vi "GenerateArmMotionProfilePoints.vi"(3 "MotionProfileGeneratorParameters":T4={"Trajectory Point Interval (ms)"=10, "Maximum Travel Speed (units/s)"=0.0, "Velocity Ramp Time (ms)"=0.0, "Acceleration Ramp Time (ms)"=1.0} {"Acceleration Ramp Time (ms)" min=1.0; "Velocity Ramp Time (ms)" min=1.0; "Maximum Travel Speed (units/s)" min=0.0; "Trajectory Point Interval (ms)" items=["TrajectoryDuration_0ms"=0, "TrajectoryDuration_5ms"=5, "TrajectoryDuration_10ms"=10, "TrajectoryDuration_20ms"=20, "TrajectoryDuration_30ms"=30, "TrajectoryDuration_40ms"=40, "TrajectoryDuration_50ms"=50, "TrajectoryDuration_100ms"=100]}, 4 "PathDistance":dbl, 5 "ArmPathIn":T1[](array[typedef]), 6 "IndexedPathLength":dbl[](array[numeric])) -> (0 "ArmPathOut":T1[](array[typedef]), 1 "ExtendPath":T2[](array[typedef]) {"Time (ms)" items=["TrajectoryDuration_0ms"=0, "TrajectoryDuration_5ms"=5, "TrajectoryDuration_10ms"=10, "TrajectoryDuration_20ms"=20, "TrajectoryDuration_30ms"=30, "TrajectoryDuration_40ms"=40, "TrajectoryDuration_50ms"=50, "TrajectoryDuration_100ms"=100]}, 2 "RotatePath":T2[](array[typedef]) {"Time (ms)" items=["TrajectoryDuration_0ms"=0, "TrajectoryDuration_5ms"=5, "TrajectoryDuration_10ms"=10, "TrajectoryDuration_20ms"=20, "TrajectoryDuration_30ms"=30, "TrajectoryDuration_40ms"=40, "TrajectoryDuration_50ms"=50, "TrajectoryDuration_100ms"=100]})   [LabVIEW 2017]
uses:
  TypeDefs/ArmCoordinate.ctl
  General/MotionProfiling/TypeDefs/MotionProfileGeneratorParams.ctl
  <vilib>/Rock Robotics/WPI/ThirdParty/Phoenix-LabVIEW/Motor Controller/Controls/CTRE_Phoenix_MotorControl_TrajectoryPointTimeDur.ctl
  General/MotionProfiling/TypeDefs/TrajectoryPoint.ctl
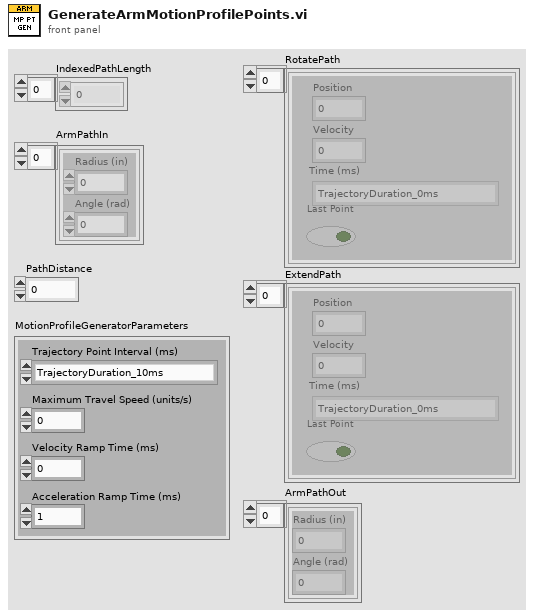
[diagram p1: front panel]
types:
  T1 = typedef "ArmCoordinate.ctl" = cluster{"Radius (in)":dbl, "Angle (rad)":dbl}
  T2 = typedef "TrajectoryPoint.ctl" = cluster{"Position ":dbl, "Velocity ":dbl, "Time (ms)":T3, "Last Point":bool}
  T3 = typedef "CTRE_Phoenix_MotorControl_TrajectoryPointTimeDur.ctl" = i32
  T4 = typedef "MotionProfileGeneratorParams.ctl" = cluster{"Trajectory Point Interval (ms)":T3, "Maximum Travel Speed (units/s)":dbl, "Velocity Ramp Time (ms)":dbl, "Acceleration Ramp Time (ms)":dbl}
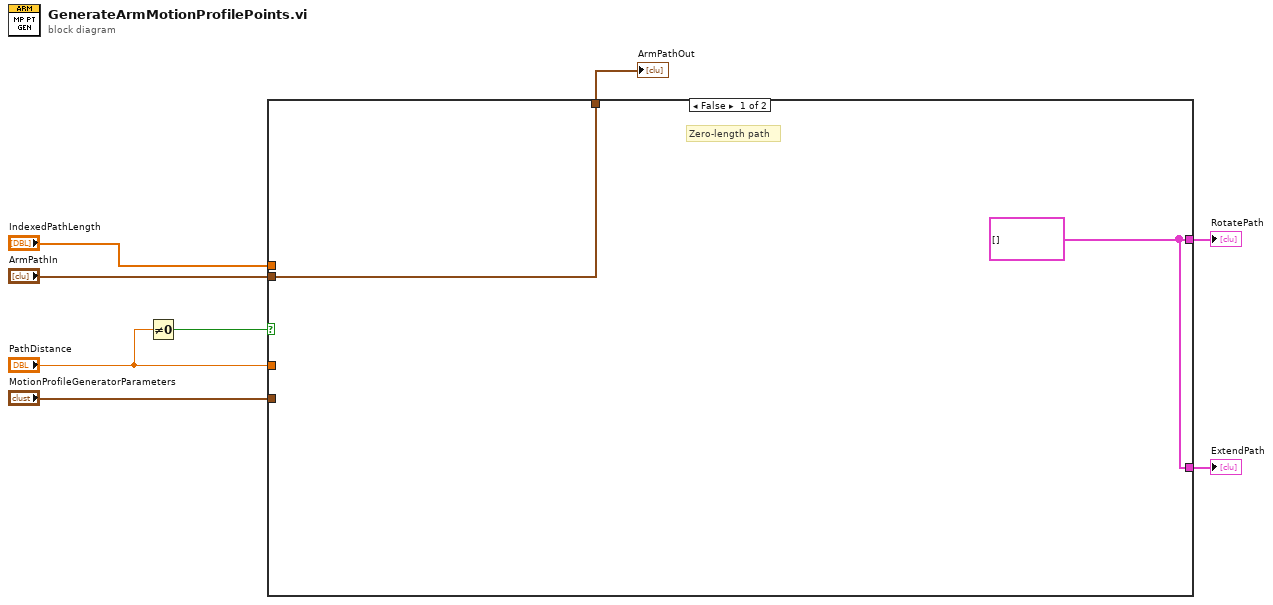
[diagram p0: block diagram]
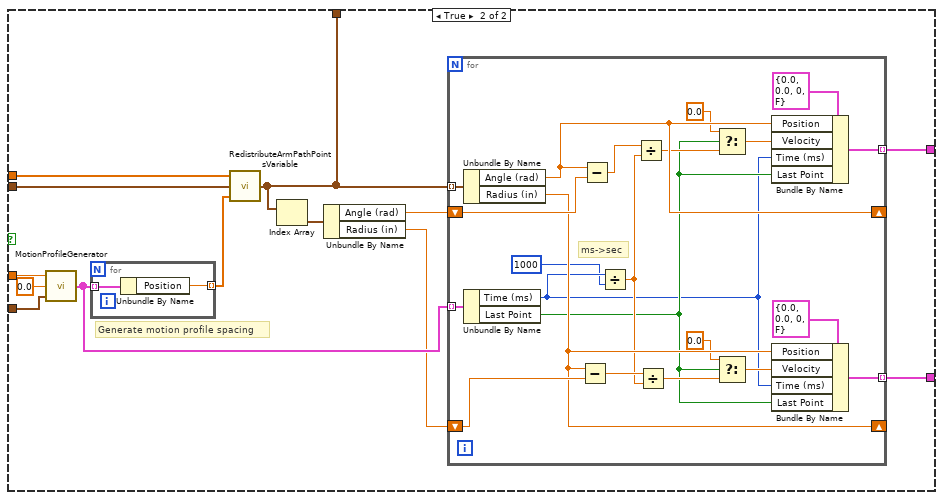
[diagram p2: hidden frame]
diagram:
  n1 = Not Equal To 0?(x="PathDistance") -> (x != 0?=w1:bool)
  n2 = case shown="False" w1 {
    tunnel: "ArmPathIn" -> [w10 w21]
    tunnel: "IndexedPathLength" -> [_ w20]
    tunnel: "MotionProfileGeneratorParameters" -> [_ w19]
    tunnel: [w9 w18] -> w5
    tunnel: [w9 w17] -> w4
    tunnel: "PathDistance" -> [_ w12]
    tunnel: [w10 w11] -> w2
    frame False {
      w9 = T2[] []
      # "Zero-length path"
    }
    frame True {
      # "Generate motion profile spacing"
      n3 = call "MotionProfileGenerator.vi"("MotionProfileGeneratorParameters"=w19, "Starting Position (units)"=0.0 ("Starting Position (rotations)"), "Travel Distance (units)"=w12) -> ("Trajectory Points"=w15:T2[])
      n4 = for {
        tunnel: w15 -> [w47] mode=indexing
        tunnel: [w46] -> w22 mode=indexing
        n5 = Unbundle By Name(w47) -> ("Position"=w46:dbl)
      }
      n6 = call "RedistributeArmPathPointsVariable.vi"("DesiredPointSpacing"=w22, "ArmPathIn"=w21, "IndexedPathLength"=w20) -> ("ArmPathOut"=w11:T1[])
      n7 = Index Array(array=w11) -> (element=w16:T1)  [unwired: 1 in]
      n8 = Unbundle By Name(w16) -> ("Angle (rad)"=w14:dbl, "Radius (in)"=w13:dbl)
      n9 = for {
        tunnel: w11 -> [w40] mode=indexing
        tunnel: w15 -> [w41] mode=indexing
        tunnel: [w43] -> w17 mode=indexing
        tunnel: [w42] -> w18 mode=indexing
        shift-right: [w38] -> _
        shift-left: w14 -> [w39]
        shift-right: [w36] -> _
        shift-left: w13 -> [w37]
        # "ms->sec"
        n10 = Unbundle By Name(w40) -> ("Angle (rad)"=w38:dbl, "Radius (in)"=w36:dbl)
        n11 = Unbundle By Name(w41) -> ("Time (ms)"=w25:T3, "Last Point"=w28:bool)
        n12 = Subtract(x=w36, y=w37) -> (x-y=w35:dbl)
        n13 = Subtract(x=w38, y=w39) -> (x-y=w34:dbl)
        n14 = Divide(x=w25, y=1000) -> (x/y=w33:dbl)
        n15 = Divide(x=w34, y=w33) -> (x/y=w32:dbl)
        n16 = Divide(x=w35, y=w33) -> (x/y=w29:dbl)
        n17 = Select(t=0.0, s=w28, f=w32) -> (s? t:f=w31:dbl)
        n18 = Select(t=0.0, s=w28, f=w29) -> (s? t:f=w27:dbl)
        n19 = Bundle By Name(cluster=T2 {"Position "=0.0, "Velocity "=0.0, "Time (ms)"=0, "Last Point"=FALSE} ("trajectory point"), "Position"=w38, "Velocity"=w31, "Time (ms)"=w25, "Last Point"=w28) -> (w42:T2)
        n20 = Bundle By Name(cluster=T2 {"Position "=0.0, "Velocity "=0.0, "Time (ms)"=0, "Last Point"=FALSE} ("trajectory point"), "Position"=w36, "Velocity"=w27, "Time (ms)"=w25, "Last Point"=w28) -> (w43:T2)
      }
    }
  }
  "RotatePath" <- w5
  "ExtendPath" <- w4
  "ArmPathOut" <- w2
